vi "Add Port.vi"(6 "speed":T1=enum."HI (100 kb/s)", 8 "error in":errorcluster, 9 "direction":T2, 10 "port number":u16, 11 "custom device ref":T3 format="%.0x") -> (0 "error out":errorcluster, 2 "port":T3 format="%.0x", 3 "custom device ref out":T3 format="%.0x")   [LabVIEW 2020, in "AIM ARINC 429 Scripting.lvlib"]
doc: "Based on the specified <b>direction</b>, adds the specified <b>port</b> to the custom device system definition. Receive (Rx) ports are added to the Ports>>Incoming subsection. Transmit (Tx) ports are added to the Ports>>Outgoing subsection. Returns the newly added <b>port</b> reference."
uses:
  AIM ARINC 429 Scripting.lvlib
  <vilib>/NI VeriStand/Custom Device API/Custom Device Item Ref.ctl
  Shared/Direction.ctl
  Shared/Transfer Speed.ctl
  Constants.vi
  <vilib>/NI VeriStand/Custom Device Tools/Custom Device Utility Library/NI VeriStand - Search for Item by GUID.vi
  <vilib>/NI VeriStand/Custom Device Tools/Custom Device Utility Library/Custom Device Utility Library.lvlib
  <vilib>/NI VeriStand/Custom Device Offline API/Custom Device Offline API.lvlib
  <vilib>/NI VeriStand/Custom Device API/Custom Device API.lvlib
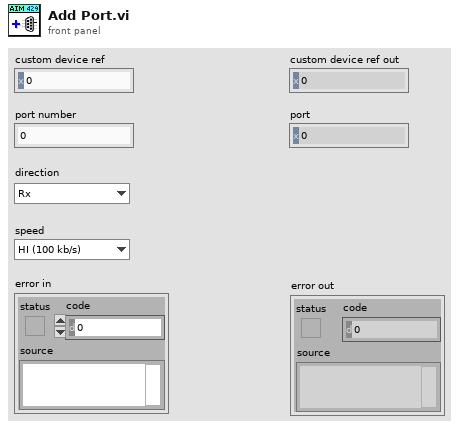
[diagram p1: front panel]
types:
  T1 = typedef "Transfer Speed.ctl" = enum16{"LO (12.5 kb/s)", "HI (100 kb/s)"}
  T2 = typedef "Direction.ctl" = enum16{"Rx", "Tx"}
  T3 = typedef "Custom Device API.lvlib/Custom Device Item Ref.ctl" = u64
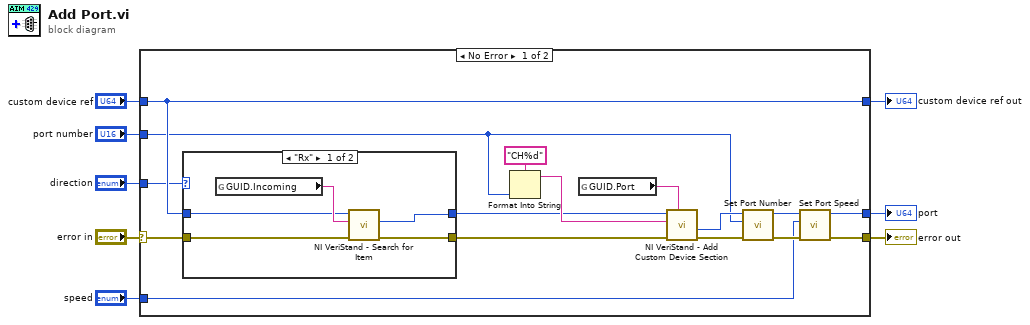
[diagram p0: block diagram]
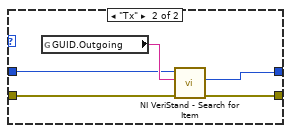
[diagram p2: hidden frame]
diagram:
  n1 = case shown="No Error" "error in" {
    selector: "error in" -> [w21 w36]
    tunnel: "custom device ref" -> [w18 w35]
    tunnel: [w10 w36] -> w7
    tunnel: [w11 _] -> w6
    tunnel: "port number" -> [w14 _]
    tunnel: [w18 w35] -> w3
    tunnel: "direction" -> [w17 _]
    tunnel: "speed" -> [w9 _]
    frame No Error {
      n2 = case shown="\"Rx\"" w17 {
        tunnel: w18 -> [w26 w32]
        tunnel: [w27 w30] -> w19
        tunnel: w21 -> [w25 w33]
        tunnel: [w28 w31] -> w20
        frame "Rx" {
          n3 = global read "Constants.vi" "GUID.Incoming"() -> (w29:string)
          n4 = call-poly <vilib>:"NI VeriStand - Search for Item.vi"("error in"=w25, "Item GUID"=w29, "Section Ref in"=w26) -> ("error out"=w28:errorcluster, "Item Ref"=w27:T3)  [unwired: 5 in, 2 out]
        }
        frame "Tx" {
          n5 = global read "Constants.vi" "GUID.Outgoing"() -> (w34:string)
          n6 = call-poly <vilib>:"NI VeriStand - Search for Item.vi"("error in"=w33, "Item GUID"=w34, "Section Ref in"=w32) -> ("error out"=w31:errorcluster, "Item Ref"=w30:T3)  [unwired: 5 in, 2 out]
        }
      }
      n7 = Format Into String(format string="CH%d", w14) -> (resulting string=w22:string)  [unwired: 2 in, 1 out]
      n8 = global read "Constants.vi" "GUID.Port"() -> (w24:string)
      n9 = call <vilib>:"NI VeriStand - Add Custom Device Section.vi"("GUID (Default Section)"=w24, "error in (no error)"=w20, "Section Name"=w22, "Parent Ref in"=w19) -> ("error out"=w16:errorcluster, "Section Ptr"=w15:T3)  [unwired: 4 in, 2 out]
      n10 = call "Set Port Number.vi"("error in"=w16, "port number"=w14, "port ref"=w15) -> ("error out"=w13:errorcluster, "port ref out"=w12:T3)  [unwired: 7 in]
      n11 = call "Set Port Speed.vi"("error in"=w13, "speed"=w9, "port ref"=w12) -> ("error out"=w10:errorcluster, "port ref out"=w11:T3)  [unwired: 7 in]
    }
    frame Error {
    }
  }
  "error out" <- w7
  "port" <- w6
  "custom device ref out" <- w3
